vi "UpdateCommandWrapperReferences.vi"() -> ()   [LabVIEW 2025]
doc: "Bordeaux: rewrites the managed command wrapper references VI in the robot target context. Deletes its Static VI References, adds one per wrapper path, records the description and saves. Refuses an unmarked VI (5001), unsaved edits (5002) and an unknown target (5003). Never runs a wrapper."
uses:
  <vilib>/Utility/traverseref.llb/VI Scripting - Traverse.lvlib
  <vilib>/Utility/traverseref.llb/TRef TravTarget.ctl
  <vilib>/Utility/miscctls.llb/LVPointTypeDef.ctl
panel:
  out "error out":errorcluster
  out "reference count":i32
  out "previous description":string
  out "context name":string
  in  "wrapper paths":string[](array[string])
  in  "marker":string
  in  "description":string
  in  "references path":string
  in  "target name":string
  in  "project path":string
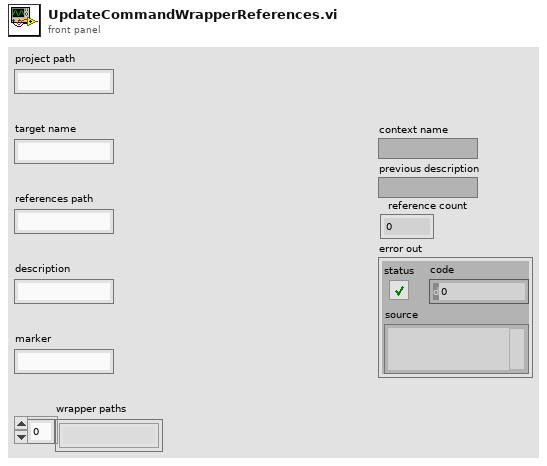
[diagram p1: front panel]
types:
  T1 = typedef "TRef TravTarget.ctl" = enum16{"FP", "BD", "Other"}
  T2 = typedef "LVPointTypeDef.ctl" = cluster{"Horizontal":i16, "Vertical":i16}
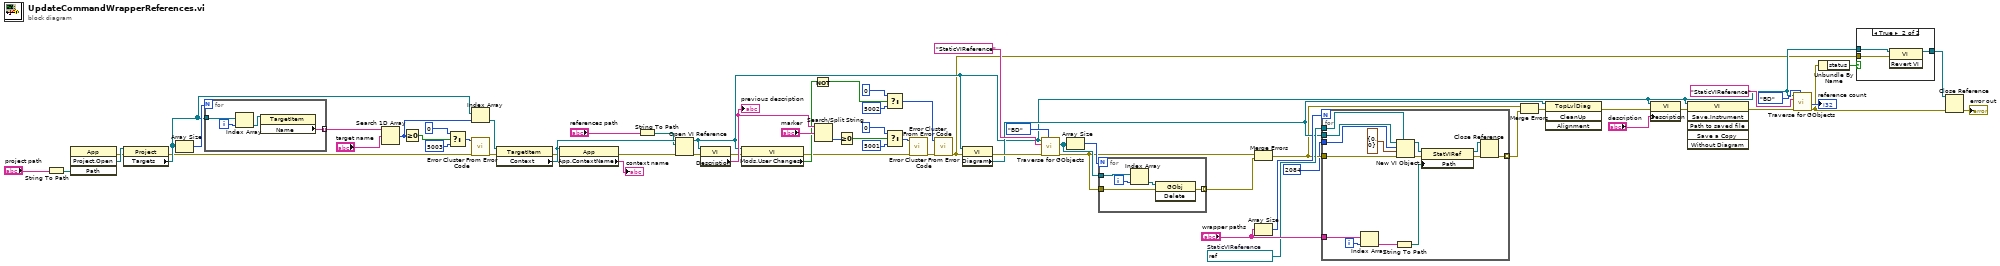
[diagram p0: block diagram]
diagram:
  w19 = refnum<vi> refnum  # StaticVIReference
  n1 = String To Path(string="project path") -> (path=w65:path)
  n2 = invoke class="App" method="Project.Open"("Path"=w65) -> (error out=w63:errorcluster, "Project:Open"=w64:refnum<vi>)  [unwired: 3 in, 2 out]
  n3 = property class="Project"(reference=w64, error in=w63) -> (error out=w53:errorcluster, "Targets"=w61:refnum<vi>[])  [unwired: 1 out]
  n4 = Array Size(array=w61) -> (size(s)=w62:i32)
  n5 = for {
    N: w62 -> [_]
    tunnel: w61 -> [w70]
    tunnel: [w67] -> w59 mode=indexing
    i -> [w69]
    n6 = Index Array(array=w70, index=w69) -> (element=w68:refnum<vi>)
    n7 = property class="TargetItem"(reference=w68) -> ("Name"=w67:string)  [unwired: 1 in, 2 out]
  }
  n8 = Search 1D Array(1D array=w59, element="target name") -> (index of element=w58:i32)  [unwired: 1 in]
  n9 = Greater Or Equal To 0?(x=w58) -> (x >= 0?=w57:bool)
  n10 = Select(t=0, s=w57, f=5003) -> (s? t:f=w54:i32)
  n11 = Index Array(array=w61, index=w58) -> (element=w52:refnum<vi>)
  n12 = call <vilib>:"Error Cluster From Error Code.vi"("error in (no error)"=w53, "error code (0)"=w54) -> ("error out"=w51:errorcluster)  [unwired: 7 in]
  n13 = property class="TargetItem"(reference=w52, error in=w51) -> (error out=w49:errorcluster, "Context"=w50:refnum<vi>)  [unwired: 1 out]
  n14 = property class="App"(reference=w50, error in=w49) -> (error out=w45:errorcluster, "App.ContextName"=→"context name":string)  [unwired: 1 out]
  n15 = String To Path(string="references path") -> (path=w46:path)
  n16 = Open VI Reference(application reference (local)=w50, vi path=w46, error in (no error)=w45) -> (vi reference=w4:refnum<vi>, error out=w44:errorcluster)  [unwired: 3 in]
  n17 = property class="VI"(reference=w4, error in=w44) -> (error out=w40:errorcluster, "Description"=w43:string)  [unwired: 1 out]
  "previous description" <- w43
  n18 = property class="VI"(reference=w4, error in=w40) -> (error out=w34:errorcluster, "Mods.User Changes"=w39:bool)  [unwired: 1 out]
  n19 = Not(x=w39) -> (.not. x?=w33:bool)
  n20 = Search/Split String(string=w43, search string/char (-)="marker") -> (offset of match=w41:i32)  [unwired: 1 in, 2 out]
  n21 = Greater Or Equal To 0?(x=w41) -> (x >= 0?=w38:bool)
  n22 = Select(t=0, s=w33, f=5002) -> (s? t:f=w30:i32)
  n23 = Select(t=0, s=w38, f=5001) -> (s? t:f=w35:i32)
  n24 = call <vilib>:"Error Cluster From Error Code.vi"("error in (no error)"=w34, "error code (0)"=w35) -> ("error out"=w29:errorcluster)  [unwired: 7 in]
  n25 = call <vilib>:"Error Cluster From Error Code.vi"("error in (no error)"=w29, "error code (0)"=w30) -> ("error out"=w3:errorcluster)  [unwired: 7 in]
  n26 = property class="VI"(reference=w4, error in=w3) -> (error out=w27:errorcluster, "Diagram"=w18:refnum<vi>)  [unwired: 1 out]
  n27 = call <vilib>:"Traverse for GObjects.vi"("Traverse Target"=TRef_TravTarget."BD", "error in (no error)"=w27, "Class Name"="StaticVIReference", "VI Refnum"=w4) -> ("error out"=w23:errorcluster, "References"=w24:refnum<vi>[])  [unwired: 4 in, 2 out]
  n28 = Array Size(array=w24) -> (size(s)=w25:i32)
  n29 = for {
    N: w25 -> [_]
    tunnel: w24 -> [w75]
    tunnel: w23 -> [w72]
    tunnel: [w71] -> w22 mode=indexing
    i -> [w74]
    n30 = Index Array(array=w75, index=w74) -> (element=w73:refnum<vi>)
    n31 = invoke class="GObj" method="Delete"(reference=w73, error in=w72) -> (error out=w71:errorcluster)  [unwired: 1 in, 2 out]
  }
  n32 = Merge Errors(w23, w22) -> (w17:errorcluster)
  n33 = Array Size(array="wrapper paths") -> (size(s)=w21:i32)
  n34 = for {
    N: w21 -> [_]
    tunnel: "wrapper paths" -> [w89]
    tunnel: w19 -> [w87]
    tunnel: w18 -> [w86]
    tunnel: w17 -> [w85]
    tunnel: u32 2084 -> [w84]
    tunnel: [w76] -> w15 mode=indexing
    i -> [w88]
    n35 = Index Array(array=w89, index=w88) -> (element=w82:string)
    n36 = String To Path(string=w82) -> (path=w79:path)
    n37 = New VI Object(vi object class=w87, owner refnum=w86, style=w84, position/next to=T2 {"Horizontal"=0, "Vertical"=0} ("location"), 8:w85) -> (object refnum=w81:refnum<vi>, 0:w80:errorcluster)  [unwired: 3 in]
    n38 = property class="StatVIRef"(reference=w81, error in=w80, "Path"=w79) -> (reference out=w78:refnum<vi>, error out=w77:errorcluster)
    n39 = Close Reference(reference=w78, error in (no error)=w77) -> (error out=w76:errorcluster)
  }
  n40 = Merge Errors(w17, w15) -> (w14:errorcluster)
  n41 = invoke class="TopLvlDiag" method="CleanUp"(reference=w18, error in=w14) -> (error out=w13:errorcluster)  [unwired: 2 in, 3 out]
  n42 = property class="VI"(reference=w4, error in=w13, "Description"="description") -> (error out=w11:errorcluster)  [unwired: 1 out]
  n43 = invoke class="VI" method="Save.Instrument"(reference=w4, error in=w11) -> (error out=w9:errorcluster)  [unwired: 4 in, 5 out]
  n44 = call <vilib>:"Traverse for GObjects.vi"("Traverse Target"=TRef_TravTarget."BD", "error in (no error)"=w9, "Class Name"="StaticVIReference", "VI Refnum"=w4) -> ("error out"=w6:errorcluster, "# of Refs"=→"reference count":i32)  [unwired: 4 in, 2 out]
  n45 = Unbundle By Name(w6) -> ("status"=w5:bool)
  n46 = case shown="True" w5 {
    tunnel: w4 -> [w90 w93]
    tunnel: w3 -> [_ w92]
    tunnel: [w90 w91] -> w2
    frame False {
    }
    frame True {
      n47 = invoke class="VI" method="Revert VI"(reference=w93, error in=w92) -> (reference out=w91:refnum<vi>)  [unwired: 1 in, 2 out]
    }
  }
  n48 = Close Reference(reference=w2, error in (no error)=w6) -> (error out=→"error out":errorcluster)
